vi "update run metadata.vi"(6 "property key-value pairs":cluster{"key":string, "value":string}[](array[cluster]), 7 "links":cluster{"title":string, "url":string}[](array[cluster]), 8 "Labels":string[](array[string]), 9 "Description":string, 10 "Title":string, 11 "run":refnum<class "Run.lvclass">) -> (0 "error out":errorcluster, 3 "updated run":refnum<class "Run.lvclass">)   [LabVIEW 2020, in "nominal core steps.lvlib"]
doc: "Updates the properties of a run, returning an updated run object. Only fields that are populated are used."
uses:
  nominal core steps.lvlib
  <vilib>/Nominal/Nominal IO Client/lv_src/Run/Run.lvclass
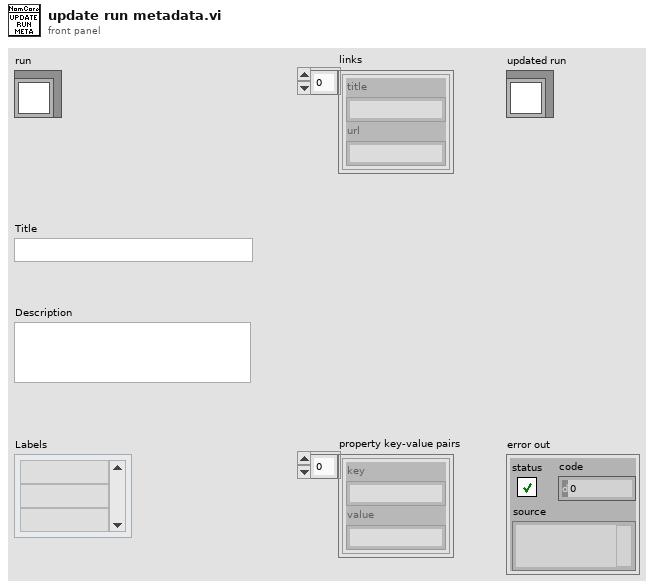
[diagram p1: front panel]
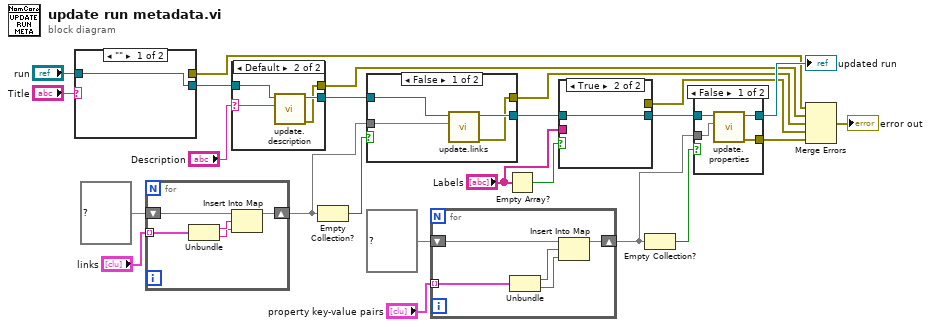
[diagram p0: block diagram]
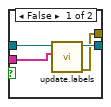
[diagram p4: hidden frame]
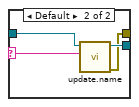
[diagram p6: hidden frame]
diagram:
  n1 = case shown="\"\"" "Title" {
    selector: "Title" -> [_ w26]
    tunnel: "run" -> [w25 w29]
    tunnel: [w25 w28] -> w23
    tunnel: [_ w27] -> w1
    frame "" {
    }
    frame Default {
      n2 = call <vilib>:"update.name.vi"("Title"=w26, "Run in"=w29) -> ("error out"=w27:errorcluster, "Run out"=w28:refnum<class "Run.lvclass">)  [unwired: 8 in]
    }
  }
  n3 = for {
    tunnel: "links" -> [w34] mode=indexing
    shift-right: [w31] -> w7
    shift-left: map{string, string} {} ("Links") -> [w32]
    n4 = Unbundle(w34) -> ("title"=w33:string, "url"=w30:string)
    n5 = Insert Into Map(map in=w32, key=w33, value=w30) -> (map out=w31:map{string, string})  [unwired: 2 out]
  }
  n6 = case shown="Default" "Description" {
    selector: "Description" -> [_ w36]
    tunnel: w23 -> [w35 w39]
    tunnel: [w35 w38] -> w22
    tunnel: [_ w37] -> w2
    frame "" {
    }
    frame Default {
      n7 = call <vilib>:"update.description.vi"("Description"=w36, "Run in"=w39) -> ("error out"=w37:errorcluster, "Run out"=w38:refnum<class "Run.lvclass">)  [unwired: 8 in]
    }
  }
  n8 = Empty Collection?(1:w7) -> (0:w10:bool)
  n9 = case shown="False" w10 {
    tunnel: w22 -> [w43 w44]
    tunnel: [w42 w44] -> w21
    tunnel: [w41 _] -> w3
    tunnel: w7 -> [w40 _]
    frame False {
      n10 = call <vilib>:"update.links.vi"("Links"=w40, "Run in"=w43) -> ("error out"=w41:errorcluster, "Run out"=w42:refnum<class "Run.lvclass">)  [unwired: 8 in]
    }
    frame True {
    }
  }
  n11 = for {
    tunnel: "property key-value pairs" -> [w49] mode=indexing
    shift-right: [w46] -> w6
    shift-left: map{string, string} {} ("map") -> [w47]
    n12 = Unbundle(w49) -> ("key"=w48:string, "value"=w45:string)
    n13 = Insert Into Map(map in=w47, key=w48, value=w45) -> (map out=w46:map{string, string})  [unwired: 2 out]
  }
  n14 = Empty Array?(array="Labels") -> (empty?=w17:bool)
  n15 = case shown="True" w17 {
    tunnel: w21 -> [w53 w54]
    tunnel: [w52 w54] -> w20
    tunnel: [w51 _] -> w4
    tunnel: "Labels" -> [w50 _]
    frame False {
      n16 = call <vilib>:"update.labels.vi"("labels"=w50, "Run in"=w53) -> ("error out"=w51:errorcluster, "Run out"=w52:refnum<class "Run.lvclass">)  [unwired: 8 in]
    }
    frame True {
    }
  }
  n17 = Empty Collection?(1:w6) -> (0:w9:bool)
  n18 = case shown="False" w9 {
    tunnel: w20 -> [w58 w59]
    tunnel: [w57 w59] -> w15
    tunnel: [w56 _] -> w14
    tunnel: w6 -> [w55 _]
    frame False {
      n19 = call <vilib>:"update.properties.vi"("properties"=w55, "Run in"=w58) -> ("error out"=w56:errorcluster, "Run out"=w57:refnum<class "Run.lvclass">)  [unwired: 8 in]
    }
    frame True {
    }
  }
  "updated run" <- w15
  n20 = Merge Errors(w1, w2, w3, w4, w14) -> (→"error out":errorcluster)
